vi "Cleanup Logs.vi"(8 "error in (no error)":errorcluster, 11 "file handler in":refnum<class "File Handler.lvclass">) -> (0 "error out":errorcluster, 3 "file handler out":refnum<class "File Handler.lvclass">)   [LabVIEW 2018, in "GLog.lvlib" / "File Handler.lvclass"]
uses:
  File Handler.lvclass
  File Handler.lvclass/File Handler.ctl
  <vilib>/Utility/error.llb/Error Cluster From Error Code.vi
  <vilib>/ErrorRing/Error Ring.xnode
  CleanupFilter/CleanupFilter.lvclass
panel:
  # "Connector Pane"
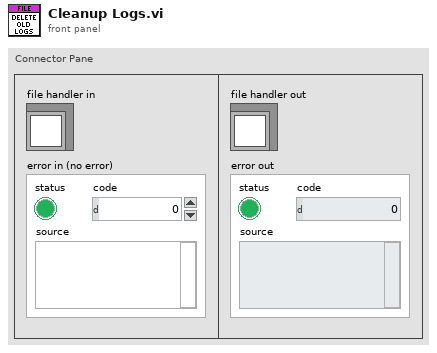
[diagram p1: front panel]
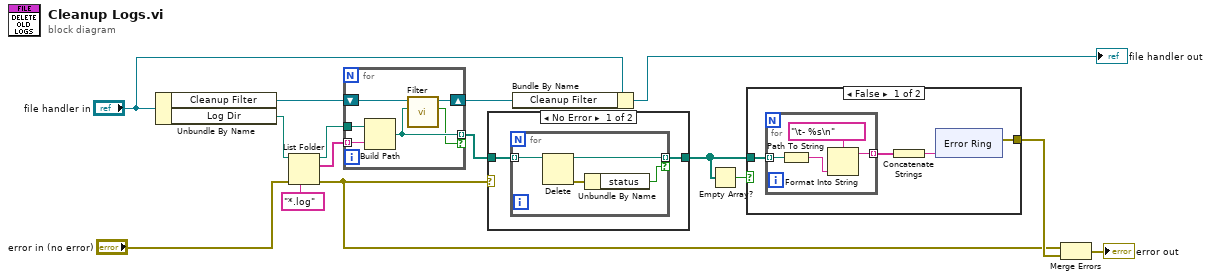
[diagram p0: block diagram]
diagram:
  n1 = Unbundle By Name("file handler in") -> ("Cleanup Filter"=w10:refnum<class "CleanupFilter.lvclass">, "Log Dir"=w15:path)
  n2 = List Folder(path=w15, pattern="*.log", error in="error in (no error)") -> (path out=w13:path, filenames=w12:string[], error out=w1:errorcluster)  [unwired: 1 in, 1 out]
  n3 = for {
    tunnel: w12 -> [w20] mode=indexing
    tunnel: w13 -> [w21]
    shift-right: [w18] -> w8
    shift-left: w10 -> [w19]
    tunnel: [w17] -> w7 mode=indexing if=w16
    n4 = Build Path(base path=w21, name or relative path=w20) -> (appended path=w17:path)
    n5 = call-dynamic "Filter.vi"("file path"=w17, "CleanupFilter in"=w19) -> ("cleanup?"=w16:bool, "CleanupFilter out"=w18:refnum<class "CleanupFilter.lvclass">)  [unwired: 8 in]
  }
  n6 = case shown="No Error" w1 {
    tunnel: w7 -> [w23 _]
    tunnel: [w22 _] -> w6
    frame No Error {
      n7 = for {
        tunnel: w23 -> [w27] mode=indexing
        tunnel: [w26] -> w22 mode=indexing if=w24
        n8 = Delete(path (use dialog)=w27) -> (deleted path=w26:path, error out=w25:errorcluster)  [unwired: 4 in, 1 out]
        n9 = Unbundle By Name(w25) -> ("status"=w24:bool)
      }
    }
    frame Error {
    }
  }
  n10 = Bundle By Name(cluster="file handler in", "Cleanup Filter"=w8) -> (→"file handler out":refnum<class "File Handler.lvclass">)
  n11 = Empty Array?(array=w6) -> (empty?=w5:bool)
  n12 = case shown="False" w5 {
    tunnel: w6 -> [w31 _]
    tunnel: [w28 _] -> w4
    frame False {
      n13 = for {
        tunnel: w31 -> [w35] mode=indexing
        tunnel: [w32] -> w30 mode=indexing
        n14 = Path To String(path=w35) -> (string=w33:string)
        n15 = Format Into String(format string="\t- %s\n", w33) -> (resulting string=w32:string)  [unwired: 2 in, 1 out]
      }
      n16 = Concatenate Strings(w30) -> (w29:string)
      n17 = xnode "Error Ring"("parameter 0"=w29) -> ("error out"=w28:errorcluster)
    }
    frame True {
    }
  }
  n18 = Merge Errors(w1, w4) -> (→"error out":errorcluster)
